vi "Sound output.vi"(5 "init":bool, 6 "error in":errorcluster, 7 "Sound Rate : rate":enum16{"11025", "22050", "44100"}(ring), 8 "sound in":dbl[](array[numeric]), 9 "Output Sound device":i32) -> (0 "error out":errorcluster, 3 "task ID out":T1 format="%.0x")   [LabVIEW 2021]
doc: "The VI write sound to a Sound Device\n\n::: CalcExpress Toolkit :::\nCopyright (c) 2000-2026 Konstantin Shifershteyn. All rights reserved."
uses:
  <vilib>/sound2/lvsound2.llb/Sound Output Task ID.ctl
  <vilib>/sound2/lvsound2.llb/Sound Data Format.ctl
  <vilib>/sound2/lvsound2.llb/Sound Output Write (DBL Single).vi
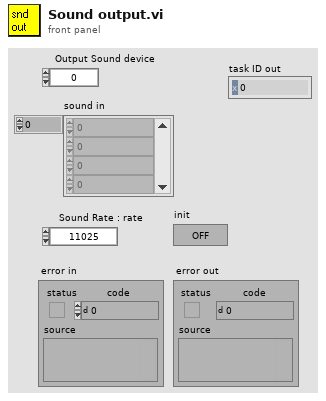
[diagram p1: front panel]
types:
  T1 = typedef "Sound Output Task ID.ctl" = u32
  T2 = typedef "Sound Data Format.ctl" = cluster{"sample rate (S/s)":dbl, "number of channels":i32, "bits per sample":i32}
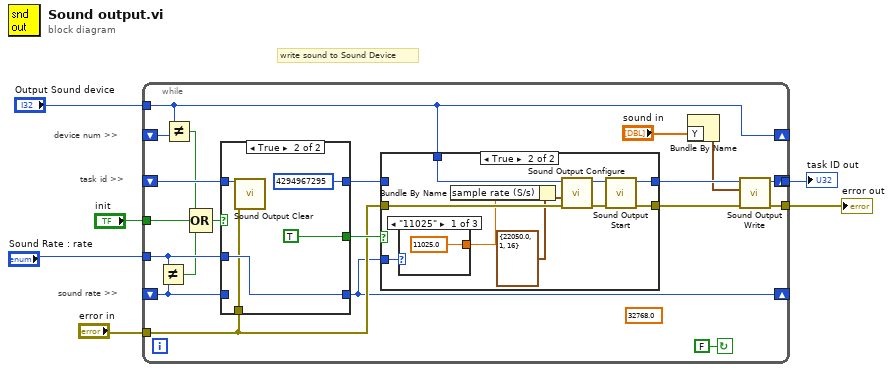
[diagram p0: block diagram]
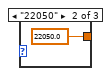
[diagram p3: hidden frame]
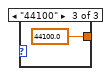
[diagram p4: hidden frame]
diagram:
  # "write sound to Sound Device"
  # "sound rate >>"
  # "task id >>"
  # "device num >>"
  n1 = while {
    tunnel: "init" -> [w13]
    tunnel: [w15] -> w3
    tunnel: "error in" -> [w17]
    tunnel: "Sound Rate : rate" -> [w23]
    shift-left: _ -> [w25]
    shift-right: [w10] -> w1
    tunnel: "Output Sound device" -> [w12]
    shift-left: _ -> [w24]
    shift-right: [w14] -> _
    shift-left: _ -> [w26]
    shift-right: [w12] -> _
    tunnel: [w10] -> _
    stop <- FALSE continue-if-true
    (unwired) 32768.0
    n2 = Not Equal?(x=w23, y=w24) -> (x != y?=w22:bool)
    n3 = Not Equal?(x=w12, y=w26) -> (x != y?=w21:bool)
    n4 = Compound Arithmetic op=OR(w21, w13, w22) -> (w20:bool)
    n5 = case shown="True" w20 {
      tunnel: w25 -> [w42 w47]
      tunnel: [w42 T1 4294967295 ("task ID out")] -> w18
      tunnel: [w43 w48] -> w14
      tunnel: w24 -> [w43 _]
      tunnel: w23 -> [_ w48]
      tunnel: [_ TRUE] -> w19
      tunnel: w17 -> [_ w45]
      frame False {
      }
      frame True {
        n6 = call <vilib>:"Sound Output Clear.vi"("error in (no error)"=w45, "task ID"=w47) -> ()  [unwired: 9 in, 1 out]
      }
    }
    n7 = case shown="True" w19 {
      tunnel: w18 -> [w28 _]
      tunnel: [w28 w36] -> w16
      tunnel: w12 -> [_ w35]
      tunnel: w17 -> [w27 w34]
      tunnel: [w27 w33] -> w9
      tunnel: w14 -> [_ w30]
      frame False {
      }
      frame True {
        n8 = case shown="\"11025\"" w30 {
          tunnel: [11025.0 22050.0 44100.0] -> w29
          frame "11025" {
          }
          frame "22050" {
          }
          frame "44100" {
          }
        }
        n9 = Bundle By Name(cluster=T2 {"sample rate (S/s)"=22050.0, "number of channels"=1, "bits per sample"=16} ("sound format"), "sample rate (S/s)"=w29) -> (w31:T2)
        n10 = call <vilib>:"Sound Output Configure.vi"("error in (no error)"=w34, "sound format"=w31, "device ID"=w35) -> ("error out"=w37:errorcluster, "task ID"=w38:T1)  [unwired: 7 in]
        n11 = call <vilib>:"Sound Output Start.vi"("error in (no error)"=w37, "task ID"=w38) -> ("error out"=w33:errorcluster, "task ID out"=w36:T1)  [unwired: 8 in]
      }
    }
    n12 = Bundle By Name("Y"="sound in") -> (w8:waveform(dbl))  [unwired: 1 in]
    n13 = call-poly <vilib>:"Sound Output Write.vi"("error in (no error)"=w9, "data"=w8, "task ID"=w16) -> ("error out"=w15:errorcluster, "task ID out"=w10:T1)  [unwired: 7 in]
  }
  "error out" <- w3
  "task ID out" <- w1
